vi "Exec Write Probe 2.vi"() -> ()   [LabVIEW 2026]
doc: "Probe: which VI execution properties VI Server can WRITE. Each write is on its own error chain; the errors come back as an array in the order of the writes."
panel:
  out "error out":errorcluster
  out "write errors":errorcluster[](array[cluster])
  in  "vi path":path
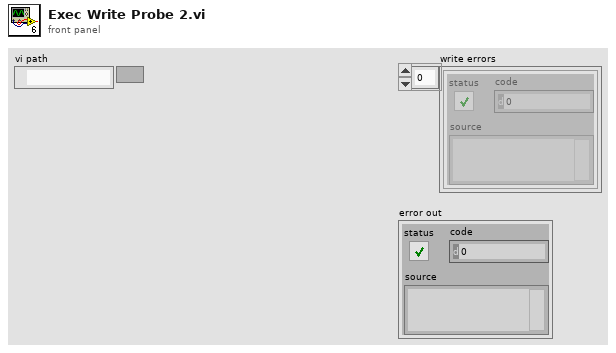
[diagram p1: front panel]
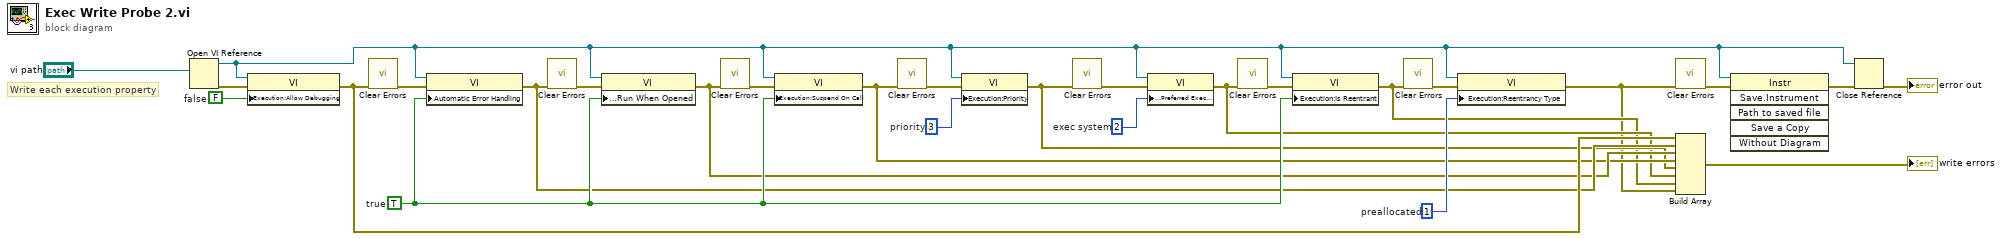
[diagram p0: block diagram]
diagram:
  w21 = u32 1  # preallocated
  w23 = 2  # exec system
  w24 = u16 3  # priority
  w22 = TRUE  # true
  w25 = FALSE  # false
  # "Write each execution property"
  n1 = Open VI Reference(vi path="vi path") -> (vi reference=w4:refnum<vi>, error out=w26:errorcluster)  [unwired: 5 in]
  n2 = property class="VI"(reference=w4, error in=w26, "Execution:Allow Debugging"=w25) -> (error out=w13:errorcluster)  [unwired: 1 out]
  n3 = call <vilib>:"Clear Errors.vi"("error in (no error)"=w13) -> ("error out"=w20:errorcluster)  [unwired: 5 in, 1 out]
  n4 = property class="VI"(reference=w4, error in=w20, "Automatic Error Handling"=w22) -> (error out=w12:errorcluster)  [unwired: 1 out]
  n5 = call <vilib>:"Clear Errors.vi"("error in (no error)"=w12) -> ("error out"=w19:errorcluster)  [unwired: 5 in, 1 out]
  n6 = property class="VI"(reference=w4, error in=w19, "Execution:Run When Opened"=w22) -> (error out=w11:errorcluster)  [unwired: 1 out]
  n7 = call <vilib>:"Clear Errors.vi"("error in (no error)"=w11) -> ("error out"=w18:errorcluster)  [unwired: 5 in, 1 out]
  n8 = property class="VI"(reference=w4, error in=w18, "Execution:Suspend On Call"=w22) -> (error out=w10:errorcluster)  [unwired: 1 out]
  n9 = call <vilib>:"Clear Errors.vi"("error in (no error)"=w10) -> ("error out"=w17:errorcluster)  [unwired: 5 in, 1 out]
  n10 = property class="VI"(reference=w4, error in=w17, "Execution:Priority"=w24) -> (error out=w9:errorcluster)  [unwired: 1 out]
  n11 = call <vilib>:"Clear Errors.vi"("error in (no error)"=w9) -> ("error out"=w16:errorcluster)  [unwired: 5 in, 1 out]
  n12 = property class="VI"(reference=w4, error in=w16, "Execution:Preferred Exec System"=w23) -> (error out=w8:errorcluster)  [unwired: 1 out]
  n13 = call <vilib>:"Clear Errors.vi"("error in (no error)"=w8) -> ("error out"=w15:errorcluster)  [unwired: 5 in, 1 out]
  n14 = property class="VI"(reference=w4, error in=w15, "Execution:Is Reentrant"=w22) -> (error out=w7:errorcluster)  [unwired: 1 out]
  n15 = call <vilib>:"Clear Errors.vi"("error in (no error)"=w7) -> ("error out"=w14:errorcluster)  [unwired: 5 in, 1 out]
  n16 = property class="VI"(reference=w4, error in=w14, "Execution:Reentrancy Type"=w21) -> (error out=w6:errorcluster)  [unwired: 1 out]
  n17 = call <vilib>:"Clear Errors.vi"("error in (no error)"=w6) -> ("error out"=w5:errorcluster)  [unwired: 5 in, 1 out]
  n18 = Build Array(w13, w12, w11, w10, w9, w8, w7, w6) -> (→"write errors":errorcluster[])
  n19 = invoke class="Instr" method="Save.Instrument"(reference=w4, error in=w5) -> (error out=w3:errorcluster)  [unwired: 4 in, 5 out]
  n20 = Close Reference(reference=w4, error in (no error)=w3) -> (error out=→"error out":errorcluster)
